vi "Test Run Suite Returns Case Results on Call to Run.vi"(8 "error in (no error)":errorcluster, 11 "Test Case In":refnum<class "LUnit Test Suite Tests.lvclass">) -> (0 "error out":errorcluster, 3 "Test Case Out":refnum<class "LUnit Test Suite Tests.lvclass">)   [LabVIEW 2020, in "LUnit Test Suite Tests.lvclass"]
uses:
  LUnit Test Suite Tests.lvclass
  LUnit Test Suite Tests.lvclass/LUnit Test Suite Tests.ctl
  source/LUnit Test Suite.lvclass
  b74e4934-f044-4222-b3dd-fc90e6c1bd4f.vi
  Test Doubles/Test Case Test Double Child/Light Test Case Double.lvclass
  source/Core/Result/Type.ctl
  source/Core/Result/Result.lvlib
  C:/git/astemes-lunit/source/Core/Runnable/Runnable.lvclass
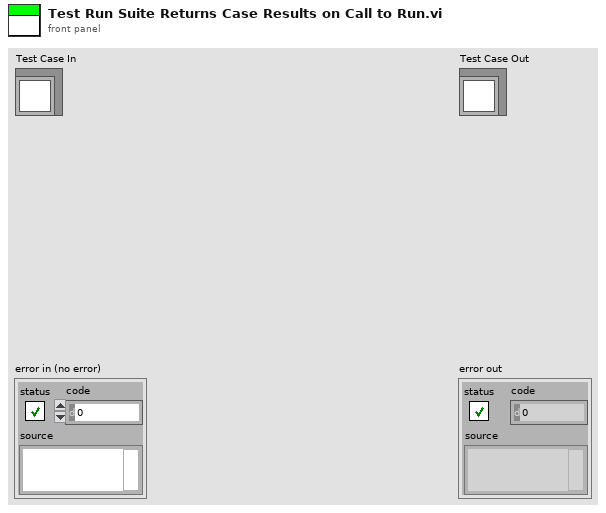
[diagram p1: front panel]
types:
  T1 = typedef "Result.lvlib/Type.ctl" = enum16{"Test Case", "Test Suite", "Test Run", "Pass", "Fail", "Skip", "Pass if", "Fail if", "Pass if Error", "Fail if Error", "Pass if Equal", "Fail if Equal"}
  T2 = typedef "Result.lvlib/Result.ctl" = cluster{"Name":string, "Description":string, "Status":T3, "Result Type":T1, "Execution Time":dbl, "Data":cluster{"Expected":variant, "Actual":variant, "Delta":variant}}
  T3 = typedef "Result.lvlib/Status.ctl" = enum16{"", "Passed", "Failed", "Error", "Skipped", "Setup Error", "Broken", "Teardown Error"}
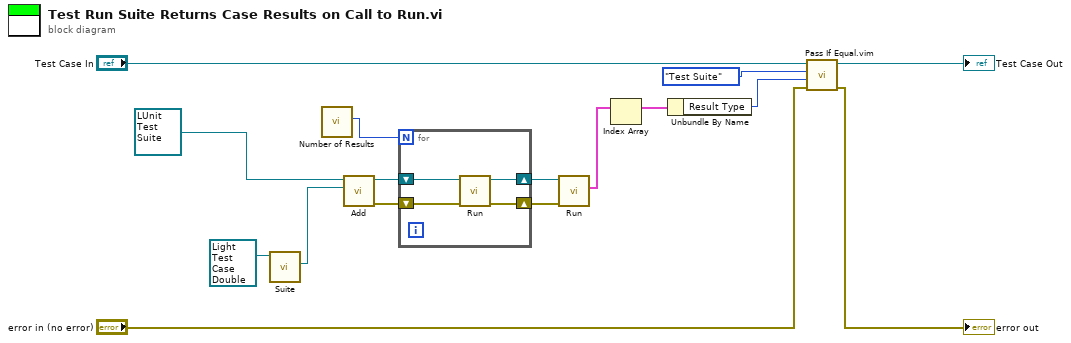
[diagram p0: block diagram]
diagram:
  n1 = call-dynamic "Suite.vi"("LUnit Test Case In"=refnum<class "Light Test Case Double.lvclass"> refnum ("LUnit Test Case V2 Test Double.lvclass")) -> ("LUnit Test Suite Out"=w9:refnum<class "LUnit Test Suite.lvclass">)  [unwired: 8 in, 2 out]
  n2 = call "Number of Results.vi"() -> ("number of methods"=w5:i32)  [unwired: 10 in, 1 out]
  n3 = call "Add.vi"("Runnable"=w9, "LUnit Test Suite In"=refnum<class "LUnit Test Suite.lvclass"> refnum ("LUnit Test Suite V2 in")) -> ("error out"=w8:errorcluster, "LUnit Test Suite Out"=w11:refnum<class "LUnit Test Suite.lvclass">)  [unwired: 8 in]
  n4 = for {
    N: w5 -> [_]
    shift-right: [w18] -> w7
    shift-left: w11 -> [w20]
    shift-right: [w17] -> w6
    shift-left: w8 -> [w19]
    n5 = call-dynamic "Run.vi"("error in (no error)"=w19, "LUnit Test Suite In"=w20) -> ("error out"=w17:errorcluster, "LUnit Test Suite In 2"=w18:refnum<class "LUnit Test Suite.lvclass">)  [unwired: 6 in, 2 out]
  }
  n6 = call-dynamic "Run.vi"("error in (no error)"=w6, "LUnit Test Suite In"=w7) -> ("Results"=w4:T2[])  [unwired: 6 in, 3 out]
  n7 = Index Array(array=w4) -> (element=w3:T2)  [unwired: 1 in]
  n8 = Unbundle By Name(w3) -> ("Result Type"=w2:T1)
  n9 = call "Pass If Equal.vim"("error in (no error)"="error in (no error)", "Actual"=w2, "Expected"=Type."Test Suite" ("Result Type"), "LUnit Test Case In"="Test Case In") -> ("error out"=→"error out":errorcluster, "LUnit Test Case Out"=→"Test Case Out":refnum<class "LUnit Test Suite Tests.lvclass">)  [unwired: 6 in]
